vi "Event Handler.vi"(0 "Tamer in":refnum<class "Tamer.lvclass">, 5 "Event type":T1=enum."Message", 7 "Item Name":string, 9 "Data":variant, 11 "error in (no error)":errorcluster) -> (4 "Tamer out":refnum<class "Tamer.lvclass">, 15 "error out":errorcluster)   [LabVIEW 2020, in "Tamer.lvlib" / "Tamer.lvclass"]
doc: "This VI is the event handler of the uService: every time an event is triggered to the uService, this VI is called.\nNote: here you can access the Actor/Class data, but it will be the one coming out from Init. You cannot modify the values.\nThree different events are supported:\nI) Button Pressed: get called on a GUI button pressed. Item Name is the name (label) of the button, Data is empty.\nII) Shared Variable Updated: get called when a SV you subscribed to is updated. Item Name is the name of the SV, and Data is the value (note: you need to convert it to the proper type).\nIII) Message: get called every time a user event is generated using Send Message to Event Handler. The values of Item Name and Data are the one given to the Send Message to Event Handler.\nIV) Ready to launch?: this frame get called every time a new Run is initiated. Each uService is responsible of performing a self check before giving back the green light for the Run to start."
uses:
  Tamer.lvclass
  TALOS/TALOS_PPL.lvlibp/Father of all uServices/Father of all uServices/Event Handler Items.ctl
  Tamer Consumer Case Selector.ctl
  TALOS/TALOS_PPL.lvlibp/Support VIs/Go-NoGo.ctl
  Run Utilities/TypeDefs/Messages/Monkey Status Message.ctl
  Run Utilities/TypeDefs/Monkey Status.ctl
  Run Utilities/Schedule/Schedule.lvclass
  Run Utilities/TypeDefs/Messages/Script Checker Message.ctl
  Run Utilities/TypeDefs/Script Checker Result.ctl
  Run Utilities/TypeDefs/Messages/Banana Message.ctl
  Run Utilities/TypeDefs/Return Code.ctl
  Tamer.lvclass/Tamer.ctl
  TALOS/TALOS_PPL.lvlibp/Guardian/Guardian/Requests.ctl
  Open Debug Window.vi
  TALOS/TALOS_PPL.lvlibp/Father of all uServices/Father of all uServices/Father of all uServices.lvclass
  TALOS/TALOS_PPL.lvlibp
  TALOS/TALOS_PPL.lvlibp/Guardian/Guardian/Guardian.lvclass
  Run Utilities/Run Utilities.lvlib
  C:/LabVIEW Code/CIRCUS/TALOS/TALOS_PPL.lvlibp/Father of all uServices/Father of all uServices/Father of all uServices.lvclass
  C:/LabVIEW Code/CIRCUS/TALOS/TALOS_PPL.lvlibp/Ancestor/Ancestor/Ancestor.lvclass
  C:/LabVIEW Code/CIRCUS/TALOS/Actor Framework.lvlibp/1abvi3w/vi.lib/ActorFramework/Actor/Actor.lvclass
  C:/LabVIEW Code/CIRCUS/CIRCUS uServices et al/Tamer/Tamer.lvclass
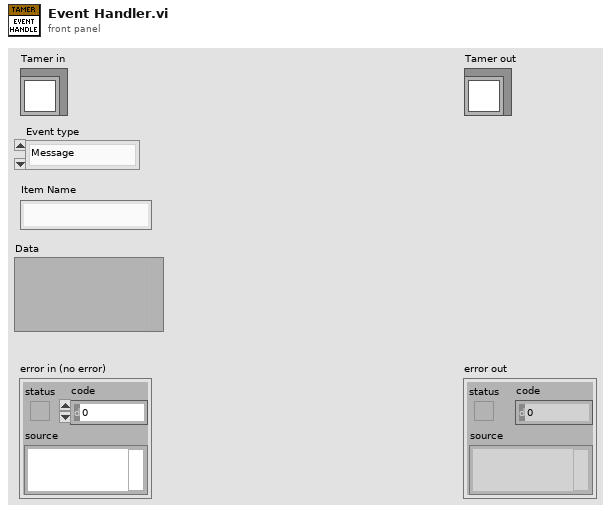
[diagram p1: front panel]
types:
  T1 = typedef "TALOS_PPL.lvlibp/Father of all uServices.lvlib/Father of all uServices.lvclass/Event Handler Items.ctl" = enum16{"Button Pressed", "Message", "Ready to launch?", "Safe Mode", "Start RUN", "Stop RUN"}
  T2 = typedef "Tamer.lvlib/Tamer.lvclass/Tamer Consumer Case Selector.ctl" = enum16{"New schedule", "Initiate RUN", "Parse Schedules", "Script Checker", "Banana after Quality Check", "Update Crit Lvl", "Propagate Banana", "Reply from Guardian", "Reply from uService", "Timeout of RUN", "uService Replies Check", "Update from Monkey", "Monkey Died", "Reschedule", "Rerun", "Stop DAQ", "Stop Schedule", "Skip Run", "Kill Process", "Update GV", "Append"}
  T3 = enum32{"Invalid", "Standard", "Closed", "Hidden", "Minimized", "Maximized"}
  T4 = typedef "TALOS_PPL.lvlibp/Go-NoGo.ctl" = cluster{"ID":string, "Status":bool, "Data":string[], "GUID":string}
  T5 = typedef "Run Utilities.lvlib/Monkey Status Message.ctl" = cluster{"Monkey ID":string, "Monkey Status":T6, "Scripts left":u32, "ETA":string, "Current Action":string, "Report from previous RUNs":string, "Skipped RUNs":refnum<class "Schedule.lvclass">}
  T6 = typedef "Run Utilities.lvlib/Monkey Status.ctl" = enum16{"Init", "Paused", "Ongoing", "Stopped", "Finished (no errors)", "Finished (with errors)"}
  T7 = typedef "Run Utilities.lvlib/Script Checker Message.ctl" = cluster{"Monkey ID":string, "Script Checker Result":T8}
  T8 = typedef "Run Utilities.lvlib/Script Checker Result.ctl" = enum16{"Passed", "Failed", "Empty"}
  T9 = typedef "Run Utilities.lvlib/Return Code.ctl" = enum16{"All Good", "Retry", "Skip", "Skip All", "ABORT"}
  T10 = typedef "Run Utilities.lvlib/Banana Message.ctl" = cluster{"FPGA Name":string, "Return Code":T9}
  T11 = typedef "TALOS_PPL.lvlibp/Guardian.lvlib/Guardian.lvclass/Requests.ctl" = enum16{"Ready to Launch", "Start RUN", "Stop RUN", "Update DAQ Params", "Update Error Listbox", "Update Run Status", "Update Kasli Log", "Run Stopped with Errors", "Switch uS View"}
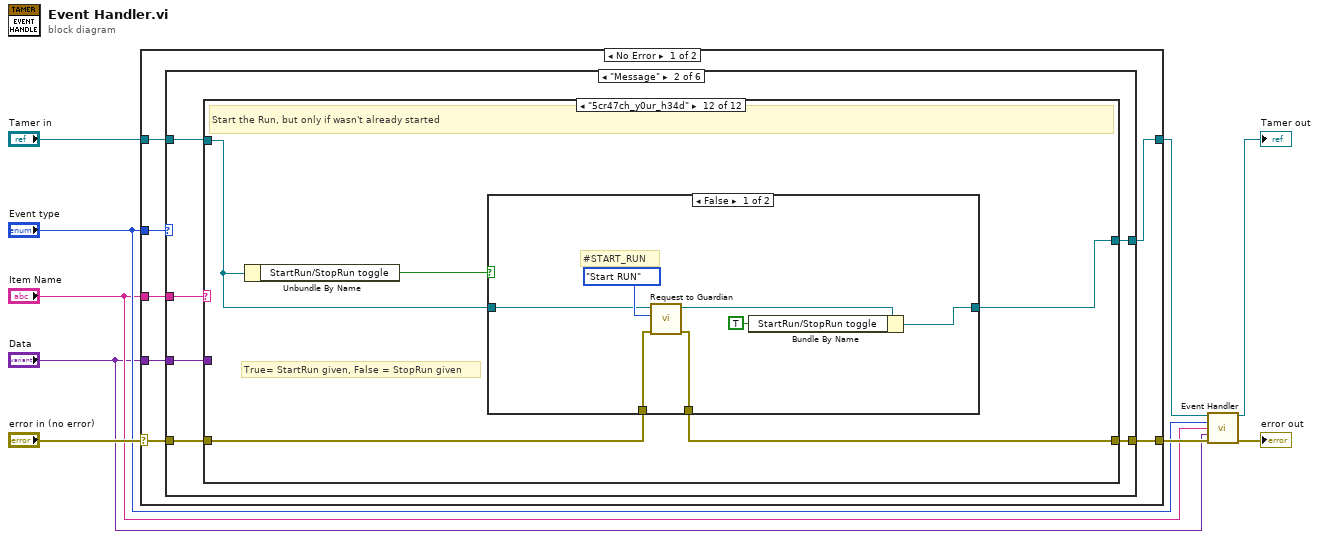
[diagram p0: block diagram]
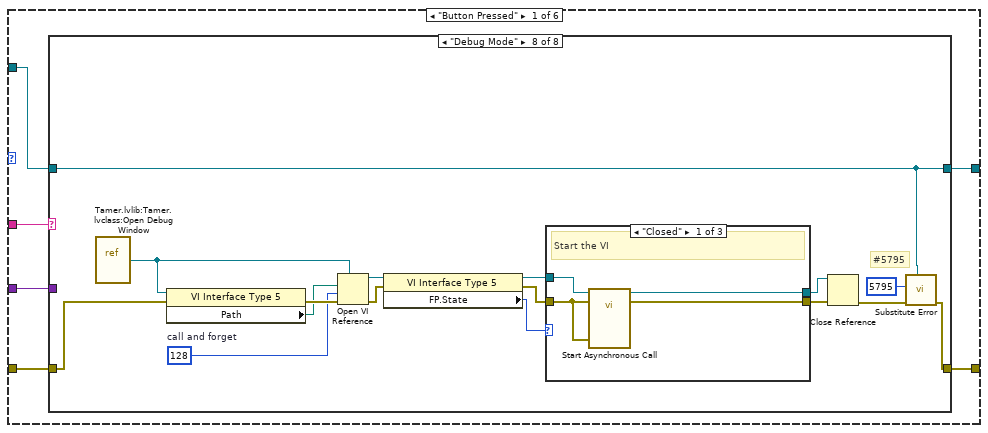
[diagram p2: hidden frame]
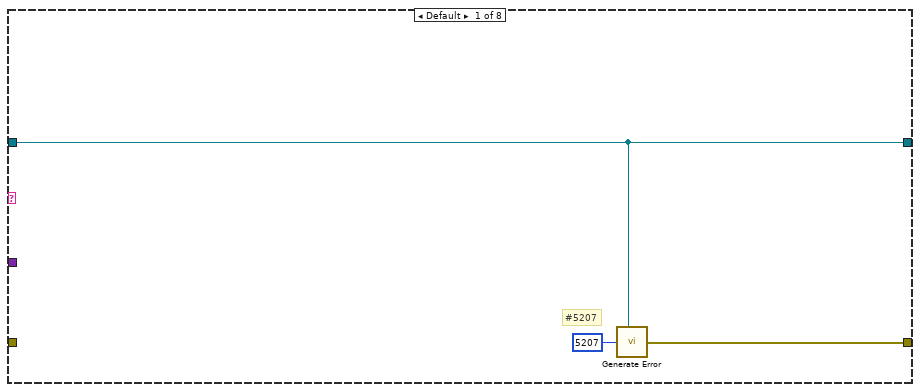
[diagram p3: hidden frame]
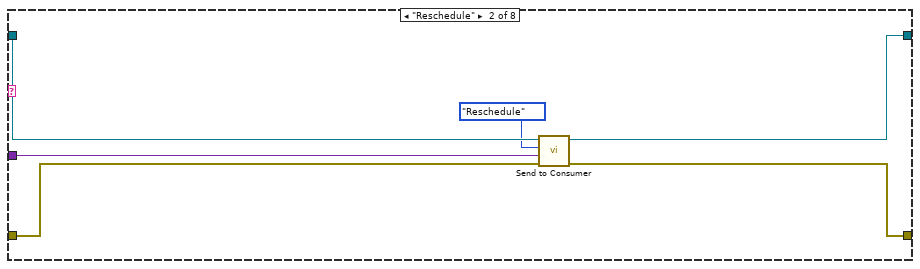
[diagram p4: hidden frame]
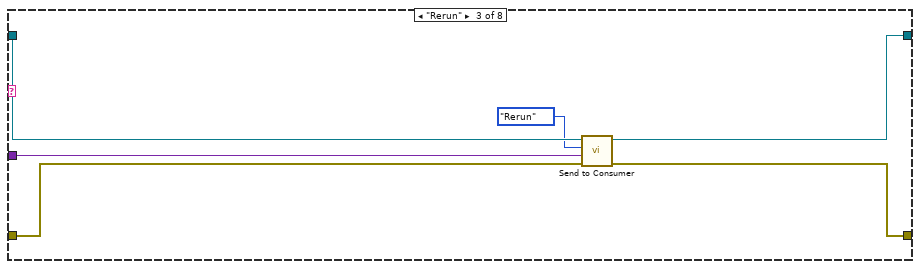
[diagram p5: hidden frame]
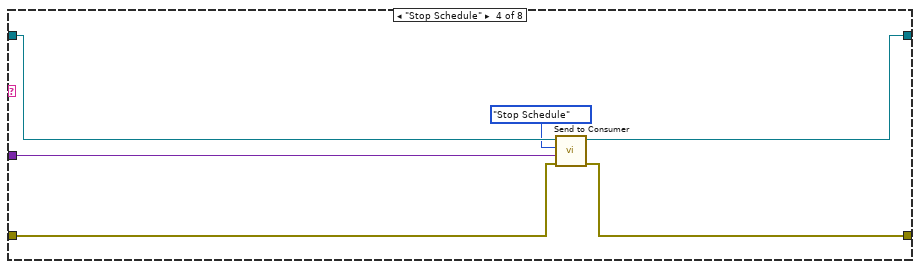
[diagram p6: hidden frame]
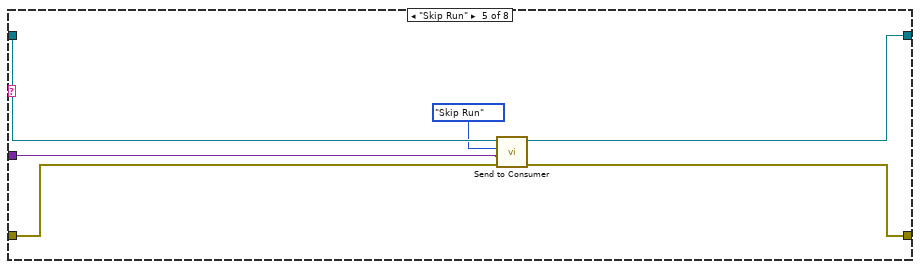
[diagram p7: hidden frame]
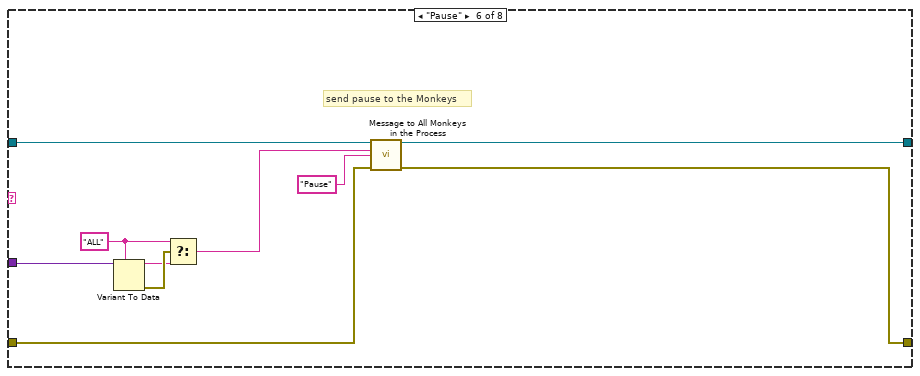
[diagram p8: hidden frame]
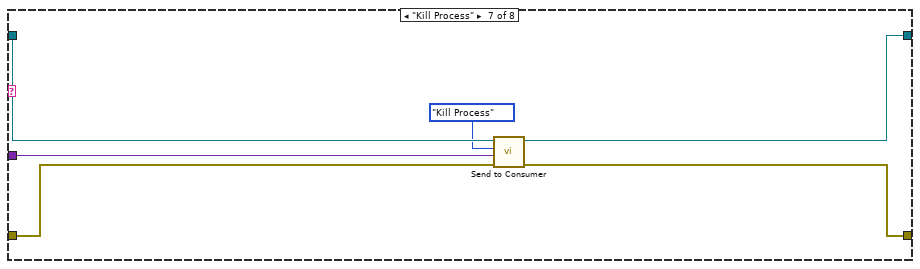
[diagram p9: hidden frame]
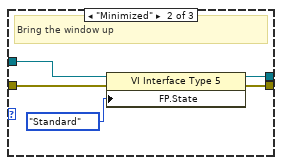
[diagram p10: hidden frame]
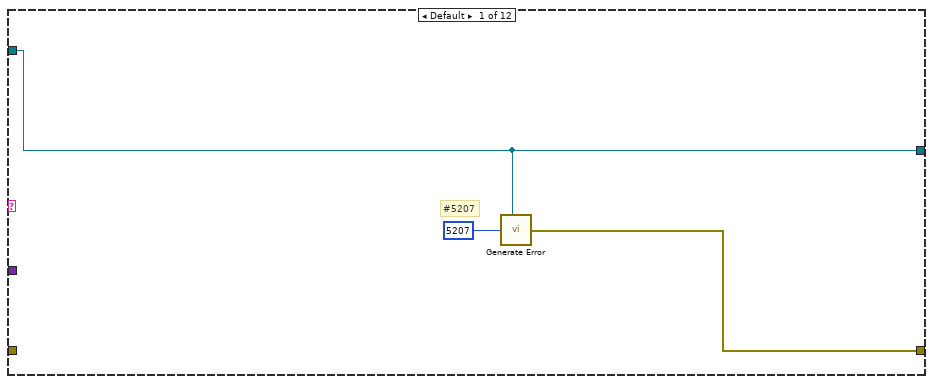
[diagram p12: hidden frame]
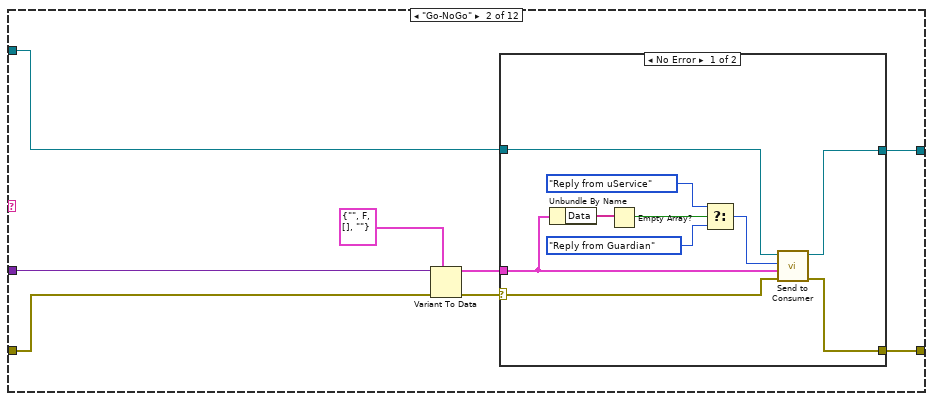
[diagram p13: hidden frame]
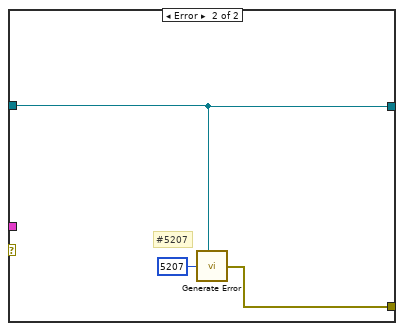
[diagram p14: hidden frame]
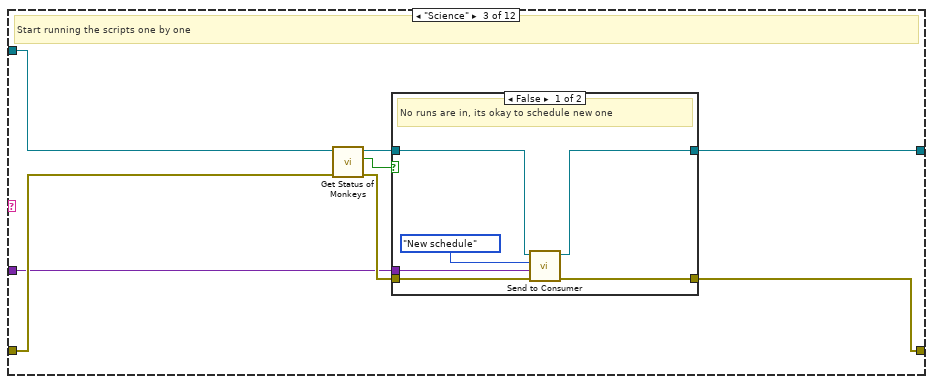
[diagram p15: hidden frame]
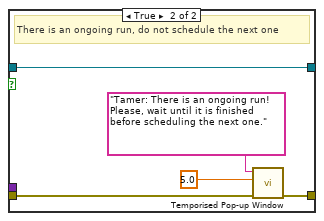
[diagram p16: hidden frame]
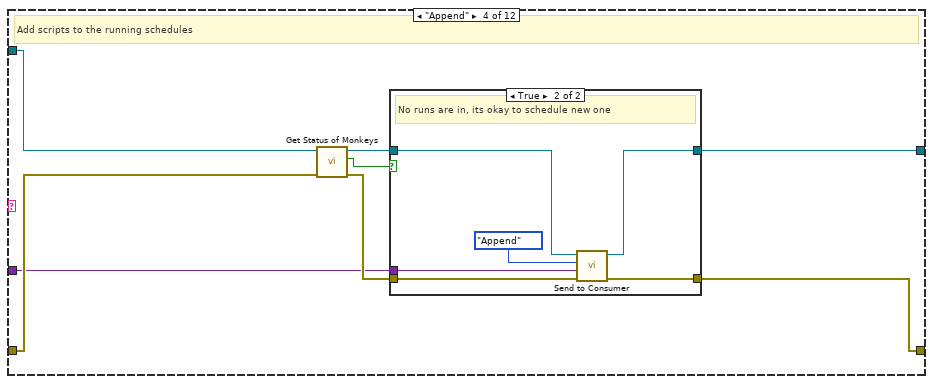
[diagram p17: hidden frame]
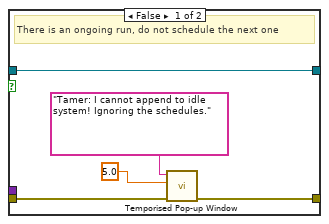
[diagram p18: hidden frame]
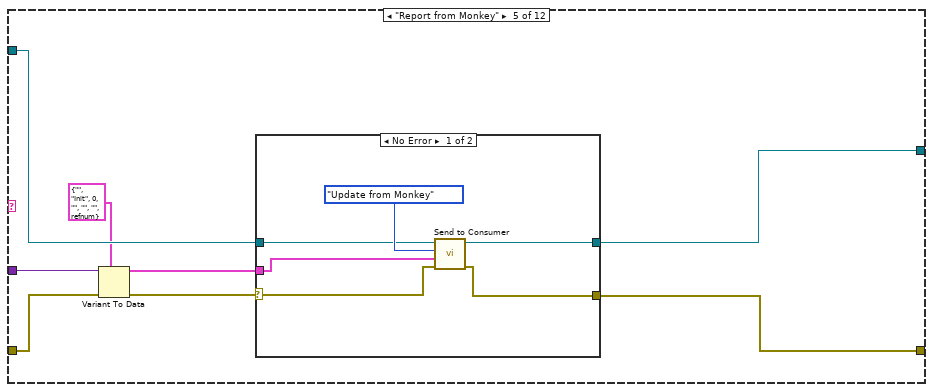
[diagram p19: hidden frame]
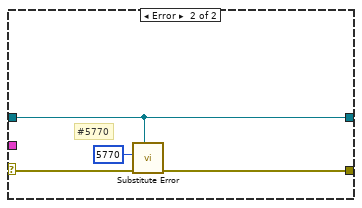
[diagram p20: hidden frame]
diagram:
  n1 = case shown="No Error" "error in (no error)" {
    selector: "error in (no error)" -> [w14 w337]
    tunnel: [w15 w337] -> w7
    tunnel: [w11 w336] -> w4
    tunnel: "Tamer in" -> [w10 w336]
    tunnel: "Event type" -> [w16 _]
    tunnel: "Item Name" -> [w13 _]
    tunnel: "Data" -> [w12 _]
    frame No Error {
      n2 = case shown="\"Message\"" w16 {
        tunnel: [w22 w94 w314 w323 w328 w335] -> w15
        tunnel: w14 -> [w19 w98 w315 w325 w329 w333]
        tunnel: w13 -> [w20 w97 _ _ _ _]
        tunnel: w10 -> [w21 w95 w313 w320 w330 w334]
        tunnel: w12 -> [w17 w96 w311 _ _ _]
        tunnel: [w18 w93 w310 w322 w326 w331] -> w11
        frame "Button Pressed" {
          n3 = case shown="\"Debug Mode\"" w20 {
            tunnel: w19 -> [_ w26 w32 w39 w45 w56 w63 w77]
            tunnel: [w24 w30 w35 w42 w46 w55 w60 w66] -> w22
            tunnel: w21 -> [w23 w31 w37 w43 w49 w58 w65 w67]
            tunnel: [w23 w28 w34 w41 w47 w57 w61 w67] -> w18
            tunnel: w17 -> [_ w27 w33 w38 w44 w54 w62 _]
            frame Default {
              # "#5207"
              n4 = call "Generate Error.vi"("Class"=w23, "Error Code"=5207) -> ("error out"=w24:errorcluster)  [unwired: 5 in]
            }
            frame "Reschedule" {
              n5 = call "Send to Consumer.vi"("error in (no error)"=w26, "Data"=w27, "Case ID"=Tamer_Consumer_Case_Selector."Reschedule" ("Monkey Consumer Case Selector"), "uService Template in"=w31) -> ("error out"=w30:errorcluster, "uService Template out"=w28:refnum<class "Tamer.lvclass">)  [unwired: 6 in]
            }
            frame "Rerun" {
              n6 = call "Send to Consumer.vi"("error in (no error)"=w32, "Data"=w33, "Case ID"=Tamer_Consumer_Case_Selector."Rerun" ("Monkey Consumer Case Selector"), "uService Template in"=w37) -> ("error out"=w35:errorcluster, "uService Template out"=w34:refnum<class "Tamer.lvclass">)  [unwired: 6 in]
            }
            frame "Stop Schedule" {
              n7 = call "Send to Consumer.vi"("error in (no error)"=w39, "Data"=w38, "Case ID"=Tamer_Consumer_Case_Selector."Stop Schedule" ("Monkey Consumer Case Selector"), "uService Template in"=w43) -> ("error out"=w42:errorcluster, "uService Template out"=w41:refnum<class "Tamer.lvclass">)  [unwired: 6 in]
            }
            frame "Skip Run" {
              n8 = call "Send to Consumer.vi"("error in (no error)"=w45, "Data"=w44, "Case ID"=Tamer_Consumer_Case_Selector."Skip Run" ("Monkey Consumer Case Selector"), "uService Template in"=w49) -> ("error out"=w46:errorcluster, "uService Template out"=w47:refnum<class "Tamer.lvclass">)  [unwired: 6 in]
            }
            frame "Pause" {
              w53 = "ALL"
              # "send pause to the Monkeys"
              n9 = Variant To Data(type=w53, Variant=w54) -> (data=w52:string, error out=w59:errorcluster)  [unwired: 1 in]
              n10 = Select(t=w53, s=w59, f=w52) -> (s? t:f=w51:string)
              n11 = call-dynamic "Message to All Monkeys in the Process.vi"("Tamer in"=w58, "Process ID"=w51, "Message"="Pause" ("Process ID"), "error in (no error)"=w56) -> ("Tamer out"=w57:refnum<class "Tamer.lvclass">, "error out"=w55:errorcluster)  [unwired: 10 in]
            }
            frame "Kill Process" {
              n12 = call "Send to Consumer.vi"("error in (no error)"=w63, "Data"=w62, "Case ID"=Tamer_Consumer_Case_Selector."Kill Process" ("Monkey Consumer Case Selector"), "uService Template in"=w65) -> ("error out"=w60:errorcluster, "uService Template out"=w61:refnum<class "Tamer.lvclass">)  [unwired: 6 in]
            }
            frame "Debug Mode" {
              w78 = 128  # call and forget
              # "#5795"
              n13 = vi-ref "Tamer.lvlib:Tamer.lvclass:Open Debug Window.vi"() -> (w76:refnum<vi>)
              n14 = property class="VI Interface Type 5"(reference=w76, error in=w77) -> (error out=w81:errorcluster, "Path"=w80:path)  [unwired: 1 out]
              n15 = Open VI Reference(type specifier VI Refnum (for type only)=w76, vi path=w80, options=w78, error in (no error)=w81) -> (vi reference=w79:refnum<vi>, error out=w74:errorcluster)  [unwired: 2 in]
              n16 = property class="VI Interface Type 5"(reference=w79, error in=w74) -> (reference out=w75:refnum<vi>, error out=w73:errorcluster, "FP.State"=w72:T3)
              n17 = case shown="\"Closed\"" w72 {
                tunnel: w75 -> [w85 w88 w92]
                tunnel: w73 -> [w84 w90 w91]
                tunnel: [w83 w89 w91] -> w69
                tunnel: [w82 w86 w92] -> w68
                frame "Closed" {
                  # "Start the VI"
                  n18 = call-by-ref "Start Asynchronous Call"(reference=w85, error in=w84, 8:"error in (no error)"=w84) -> (reference out=w82:refnum<vi>, error out=w83:errorcluster)  [unwired: 10 in, 1 out]
                }
                frame "Minimized" {
                  # "Bring the window up"
                  n19 = property class="VI Interface Type 5"(reference=w88, error in=w90, "FP.State"=T3."Standard" ("Front Panel Window:State")) -> (reference out=w86:refnum<vi>, error out=w89:errorcluster)
                }
                frame Default {
                  # "Either running or something is worng, do nothing"
                }
              }
              n20 = Close Reference(reference=w68, error in (no error)=w69) -> (error out=w71:errorcluster)
              n21 = call "Substitute Error.vi"("LabVIEW Object"=w67, "error in (no error)"=w71, "Error Code"=5795) -> ("error out"=w66:errorcluster)  [unwired: 8 in]
            }
          }
        }
        frame "Message" {
          n22 = case shown="\"5cr47ch_y0ur_h34d\"" w97 {
            tunnel: w98 -> [_ w108 w130 w149 w167 w180 w191 w208 w246 w266 w283 w300]
            tunnel: w96 -> [_ w105 w128 w147 w168 w181 w190 w210 w242 w265 w288 _]
            tunnel: w95 -> [w99 w103 w126 w142 w165 w184 w187 w204 w247 w264 w285 w297]
            tunnel: [w100 w109 w127 w146 w162 w183 w185 w205 w243 w267 w278 w299] -> w94
            tunnel: [w99 w102 w123 w143 w161 w179 w186 w203 w252 w263 w286 w298] -> w93
            frame Default {
              # "#5207"
              n23 = call "Generate Error.vi"("Class"=w99, "Error Code"=5207) -> ("error out"=w100:errorcluster)  [unwired: 5 in]
            }
            frame "Go-NoGo" {
              n24 = Variant To Data(error in=w108, type=T4 {"ID"="", "Status"=FALSE, "Data"=[], "GUID"=""} ("Go-NoGo"), Variant=w105) -> (data=w104:T4, error out=w106:errorcluster)
              n25 = case shown="No Error" w106 {
                selector: w106 -> [w117 _]
                tunnel: [w119 w121] -> w109
                tunnel: w104 -> [w114 _]
                tunnel: w103 -> [w116 w120]
                tunnel: [w115 w120] -> w102
                frame No Error {
                  n26 = Unbundle By Name(w114) -> ("Data"=w118:string[])
                  n27 = Empty Array?(array=w118) -> (empty?=w113:bool)
                  n28 = Select(t=Tamer_Consumer_Case_Selector."Reply from uService" ("Monkey Consumer Case Selector"), s=w113, f=Tamer_Consumer_Case_Selector."Reply from Guardian" ("Monkey Consumer Case Selector")) -> (s? t:f=w110:T2)
                  n29 = call "Send to Consumer.vi"("error in (no error)"=w117, "Data"=w114, "Case ID"=w110, "uService Template in"=w116) -> ("error out"=w119:errorcluster, "uService Template out"=w115:refnum<class "Tamer.lvclass">)  [unwired: 6 in]
                }
                frame Error {
                  # "#5207"
                  n30 = call "Generate Error.vi"("Class"=w120, "Error Code"=5207) -> ("error out"=w121:errorcluster)  [unwired: 5 in]
                }
              }
            }
            frame "Science" {
              # "Start running the scripts one by one"
              n31 = call-dynamic "Get Status of Monkeys.vi"("error in (no error)"=w130, "Tamer in"=w126) -> ("error out"=w129:errorcluster, "Anything running?"=w124:bool, "Tamer out"=w125:refnum<class "Tamer.lvclass">)  [unwired: 7 in]
              n32 = case shown="False" w124 {
                tunnel: w128 -> [w134 _]
                tunnel: [w136 w138] -> w127
                tunnel: w125 -> [w131 w137]
                tunnel: w129 -> [w133 w141]
                tunnel: [w132 w137] -> w123
                frame False {
                  # "No runs are in, its okay to schedule new one"
                  n33 = call "Send to Consumer.vi"("error in (no error)"=w133, "Data"=w134, "Case ID"=Tamer_Consumer_Case_Selector."New schedule" ("Monkey Consumer Case Selector"), "uService Template in"=w131) -> ("error out"=w136:errorcluster, "uService Template out"=w132:refnum<class "Tamer.lvclass">)  [unwired: 6 in]
                }
                frame True {
                  # "There is an ongoing run, do not schedule the next one"
                  n34 = call "Temporised Pop-up Window.vi"("error in (no error)"=w141, "Timeout"=5.0, "Text"="Tamer: There is an ongoing run! Please, wait until it is finished before scheduling the next one.") -> ("error out"=w138:errorcluster)  [unwired: 8 in]
                }
              }
            }
            frame "Append" {
              # "Add scripts to the running schedules"
              n35 = call-dynamic "Get Status of Monkeys.vi"("error in (no error)"=w149, "Tamer in"=w142) -> ("error out"=w148:errorcluster, "Anything running?"=w144:bool, "Tamer out"=w145:refnum<class "Tamer.lvclass">)  [unwired: 7 in]
              n36 = case shown="True" w144 {
                tunnel: w147 -> [_ w157]
                tunnel: [w151 w159] -> w146
                tunnel: w145 -> [w150 w160]
                tunnel: w148 -> [w154 w156]
                tunnel: [w150 w155] -> w143
                frame False {
                  # "There is an ongoing run, do not schedule the next one"
                  n37 = call "Temporised Pop-up Window.vi"("error in (no error)"=w154, "Timeout"=5.0, "Text"="Tamer: I cannot append to idle system! Ignoring the schedules.") -> ("error out"=w151:errorcluster)  [unwired: 8 in]
                }
                frame True {
                  # "No runs are in, its okay to schedule new one"
                  n38 = call "Send to Consumer.vi"("error in (no error)"=w156, "Data"=w157, "Case ID"=Tamer_Consumer_Case_Selector."Append" ("Monkey Consumer Case Selector"), "uService Template in"=w160) -> ("error out"=w159:errorcluster, "uService Template out"=w155:refnum<class "Tamer.lvclass">)  [unwired: 6 in]
                }
              }
            }
            frame "Report from Monkey" {
              n39 = Variant To Data(error in=w167, type=T5 {"Monkey ID"="", "Monkey Status"=enum."Init", "Scripts left"=0, "ETA"="", "Current Action"="", "Report from previous RUNs"="", "Skipped RUNs"=refnum} ("Monkey Status Message"), Variant=w168) -> (data=w164:T5, error out=w166:errorcluster)
              n40 = case shown="No Error" w166 {
                selector: w166 -> [w173 w178]
                tunnel: w165 -> [w172 w175]
                tunnel: w164 -> [w171 _]
                tunnel: [w170 w176] -> w162
                tunnel: [w169 w175] -> w161
                frame No Error {
                  n41 = call "Send to Consumer.vi"("error in (no error)"=w173, "Data"=w171, "Case ID"=Tamer_Consumer_Case_Selector."Update from Monkey" ("Monkey Consumer Case Selector"), "uService Template in"=w172) -> ("error out"=w170:errorcluster, "uService Template out"=w169:refnum<class "Tamer.lvclass">)  [unwired: 6 in]
                }
                frame Error {
                  # "#5770"
                  n42 = call "Substitute Error.vi"("LabVIEW Object"=w175, "error in (no error)"=w178, "Error Code"=5770) -> ("error out"=w176:errorcluster)  [unwired: 8 in]
                }
              }
            }
            frame "I'm DEAD" {
              # "Monkey was killed with the STOP button (or harakiri)"
              n43 = call "Send to Consumer.vi"("error in (no error)"=w180, "Data"=w181, "Case ID"=Tamer_Consumer_Case_Selector."Monkey Died" ("Monkey Consumer Case Selector"), "uService Template in"=w184) -> ("error out"=w183:errorcluster, "uService Template out"=w179:refnum<class "Tamer.lvclass">)  [unwired: 6 in]
            }
            frame "Script Checker" {
              # "Synced Monkey Performed Script Check"
              n44 = Variant To Data(error in=w191, type=T7 {"Monkey ID"="", "Script Checker Result"=enum."Passed"} ("Message"), Variant=w190) -> (data=w188:T7, error out=w189:errorcluster)
              n45 = case shown="No Error" w189 {
                selector: w189 -> [w194 w200]
                tunnel: [w198 w201] -> w185
                tunnel: w187 -> [w197 w199]
                tunnel: w188 -> [w196 _]
                tunnel: [w193 w199] -> w186
                frame No Error {
                  n46 = call "Send to Consumer.vi"("error in (no error)"=w194, "Data"=w196, "Case ID"=Tamer_Consumer_Case_Selector."Script Checker" ("Monkey Consumer Case Selector"), "uService Template in"=w197) -> ("error out"=w198:errorcluster, "uService Template out"=w193:refnum<class "Tamer.lvclass">)  [unwired: 6 in]
                }
                frame Error {
                  # "#5757"
                  n47 = call "Substitute Error.vi"("LabVIEW Object"=w199, "error in (no error)"=w200, "Error Code"=5757) -> ("error out"=w201:errorcluster)  [unwired: 8 in]
                }
              }
            }
            frame "B4n4n4" {
              # "Script finished. Send it to Monkey for the quality check"
              n48 = Variant To Data(error in=w208, type=string[] [], Variant=w210) -> (data=w207:string[], error out=w206:errorcluster)
              n49 = case shown="No Error" w206 {
                selector: w206 -> [w233 w241]
                tunnel: w207 -> [w237 _]
                tunnel: [w217 w240] -> w205
                tunnel: w204 -> [w231 w238]
                tunnel: [w228 w238] -> w203
                frame No Error {
                  w211 = "Quality Check" ("Message")
                  # "#5752\nB4n4n4"
                  n50 = Index Array(array=w237) -> (element #1=w218:string, element #2=w234:string)  [unwired: 2 in]
                  n51 = Decimal String To Number(string=w234, default (0L)=3) -> (number=w235:i32)  [unwired: 1 in, 1 out]
                  n52 = Variant To Data(error in=w233, type=Return_Code."Skip All" ("Return Code"), Variant=w235) -> (data=w227:T9, error out=w230:errorcluster)
                  n53 = call-dynamic "Get Monkey ID From FPGA Name.vi"("error in (no error)"=w230, "FPGA Name"=w218, "Tamer in"=w231) -> ("error out"=w226:errorcluster, "Monkey ID"=w221:string, "Tamer out"=w225:refnum<class "Tamer.lvclass">)  [unwired: 6 in]
                  n54 = Bundle(cluster=T10 {"FPGA Name"="", "Return Code"=enum."All Good"} ("Cluster"), "FPGA Name"=w218, "Return Code"=w227) -> (w216:T10)
                  n55 = call "Message to uService.vi"("Father of all uServices in"=w225, "uService ID"=w221, "Message"=w211, "Data"=w216, "error in (no error)"=w226) -> ("Father of all uServices out"=w215:refnum<class "Tamer.lvclass">, "error out"=w222:errorcluster)  [unwired: 9 in]
                  n56 = Concatenate Strings(w211, " to " ("string"), w221) -> (w220:string)
                  n57 = call "FPGA informative error on return.vi"("Message"=w216, "Class in"=w215) -> ("error out"=w213:errorcluster)  [unwired: 9 in]
                  n58 = call-dynamic "Update Action History.vi"("error in (no error)"=w222, "Action"=w220, "Tamer in"=w215) -> ("error out"=w214:errorcluster, "Tamer out"=w228:refnum<class "Tamer.lvclass">)  [unwired: 7 in]
                  n59 = Merge Errors(w214, w213) -> (w212:errorcluster)
                  n60 = call "Substitute Error.vi"("LabVIEW Object"=w228, "error in (no error)"=w212, "Error Code"=5752, "Optional String"="Tamer doesn't know who sent B4n4n4") -> ("error out"=w217:errorcluster)  [unwired: 7 in]
                }
                frame Error {
                  # "#5789"
                  n61 = call "Substitute Error.vi"("LabVIEW Object"=w238, "error in (no error)"=w241, "Error Code"=5789) -> ("error out"=w240:errorcluster)  [unwired: 8 in]
                }
              }
            }
            frame "Quality Check - result" {
              n62 = Variant To Data(type=T10 {"FPGA Name"="", "Return Code"=enum."All Good"} ("Cluster"), Variant=w242) -> (data=w248:T10, error out=w249:errorcluster)  [unwired: 1 in]
              n63 = case shown="No Error" w249 {
                tunnel: w248 -> [w257 _]
                tunnel: w247 -> [w260 w261]
                tunnel: [w255 _] -> w244
                tunnel: [w256 w261] -> w253
                frame No Error {
                  # "Check if quality of run was passed. If not, give an error to have that information in the error log"
                  n64 = Unbundle By Name(w257) -> ("FPGA Name"=w258:string)
                  n65 = Concatenate Strings("Received the quality check from ", w258) -> (w254:string)
                  n66 = call-dynamic "Update Action History.vi"("Action"=w254, "Tamer in"=w260) -> ("error out"=w255:errorcluster, "Tamer out"=w256:refnum<class "Tamer.lvclass">)  [unwired: 8 in]
                }
                frame Error {
                  # "Wrong format, this is delt with in the consumer"
                }
              }
              n67 = call "Send to Consumer.vi"("error in (no error)"=w246, "Data"=w242, "Case ID"=Tamer_Consumer_Case_Selector."Banana after Quality Check" ("Monkey Consumer Case Selector"), "uService Template in"=w253) -> ("error out"=w245:errorcluster, "uService Template out"=w252:refnum<class "Tamer.lvclass">)  [unwired: 6 in]
              n68 = Merge Errors(w245, w244) -> (w243:errorcluster)
            }
            frame "570prun" {
              # "True= StartRun given, False = StopRun given"
              # "Issue Stop Run to all the uServices and Guardians."
              n69 = Unbundle By Name(w264) -> ("StartRun/StopRun toggle"=w262:bool)
              n70 = case shown="True" w262 {
                tunnel: [w269 w277] -> w267
                tunnel: w266 -> [w269 w276]
                tunnel: w265 -> [_ w275]
                tunnel: w264 -> [w268 w273]
                tunnel: [w268 w271] -> w263
                frame False {
                  # "Do nothing"
                }
                frame True {
                  # "#STOP_RUN"
                  n71 = call "Request to Guardian.vi"("error in (no error)"=w276, "Data"=w275, "Requests"=Requests."Stop RUN", "Father of all uServices in"=w273) -> ("error out"=w277:errorcluster, "Father of all uServices out"=w272:refnum<class "Tamer.lvclass">)  [unwired: 6 in]
                  n72 = Bundle By Name(cluster=w272, "StartRun/StopRun toggle"=FALSE) -> (w271:refnum<class "Tamer.lvclass">)
                }
              }
            }
            frame "Error Criticality" {
              # "Error occured when running a script"
              n73 = call-dynamic "Get Status of Monkeys.vi"("error in (no error)"=w283, "Tamer in"=w285) -> ("error out"=w289:errorcluster, "Anything running?"=w281:bool, "Tamer out"=w284:refnum<class "Tamer.lvclass">)  [unwired: 7 in]
              n74 = Not(x=w289) -> (.not. x?=w282:bool)
              n75 = Select(t=w281, s=w282, f=TRUE) -> (s? t:f=w279:bool)
              n76 = case shown="True" w279 {
                tunnel: w288 -> [_ w294]
                tunnel: [_ w293] -> w287
                tunnel: [w290 w291] -> w286
                tunnel: w284 -> [w290 w295]
                frame False {
                }
                frame True {
                  n77 = call "Send to Consumer.vi"("Data"=w294, "Case ID"=Tamer_Consumer_Case_Selector."Update Crit Lvl" ("Monkey Consumer Case Selector"), "uService Template in"=w295) -> ("error out"=w293:errorcluster, "uService Template out"=w291:refnum<class "Tamer.lvclass">)  [unwired: 7 in]
                }
              }
              n78 = Merge Errors(w287, w289) -> (w278:errorcluster)
            }
            frame "5cr47ch_y0ur_h34d" {
              # "True= StartRun given, False = StopRun given"
              # "Start the Run, but only if wasn't already started"
              n79 = Unbundle By Name(w297) -> ("StartRun/StopRun toggle"=w296:bool)
              n80 = case shown="False" w296 {
                tunnel: w300 -> [w307 w308]
                tunnel: [w306 w308] -> w299
                tunnel: [w303 w309] -> w298
                tunnel: w297 -> [w301 w309]
                frame False {
                  # "#START_RUN"
                  n81 = call "Request to Guardian.vi"("error in (no error)"=w307, "Requests"=Requests."Start RUN", "Father of all uServices in"=w301) -> ("error out"=w306:errorcluster, "Father of all uServices out"=w305:refnum<class "Tamer.lvclass">)  [unwired: 7 in]
                  n82 = Bundle By Name(cluster=w305, "StartRun/StopRun toggle"=TRUE ("StartRun already given?")) -> (w303:refnum<class "Tamer.lvclass">)
                }
                frame True {
                  # "Do nothing"
                }
              }
            }
          }
        }
        frame "Ready to launch?" {
          # "Don't remove this wire!"
          # "Just give green light: \"Cogito ergo sum\" - Volpe"
          n83 = call-dynamic "Go-NoGo.vi"("error in (no error)"=w315, "Go-NoGo Data"=w311, "Go?"=TRUE, "Father of all uServices in"=w313) -> ("error out"=w314:errorcluster, "Father of all uServices out"=w310:refnum<class "Tamer.lvclass">)  [unwired: 6 in]
        }
        frame "Safe Mode" {
          n84 = call-dynamic "Update Monkeys Status.vi"("In ALL?"=TRUE, "Status"=Monkey_Status."Finished (with errors)", "Tamer in"=w320) -> ("error out"=w318:errorcluster, "Tamer out"=w321:refnum<class "Tamer.lvclass">)  [unwired: 7 in]
          n85 = call "Send to Consumer.vi"("Case ID"=Tamer_Consumer_Case_Selector."Stop Schedule" ("Monkey Consumer Case Selector"), "uService Template in"=w321) -> ("error out"=w319:errorcluster, "uService Template out"=w322:refnum<class "Tamer.lvclass">)  [unwired: 8 in]
          n86 = Merge Errors(w319, w318, w325) -> (w323:errorcluster)
        }
        frame "Start RUN" {
          n87 = call-dynamic "Update Action History.vi"("error in (no error)"=w329, "Action"="Start Run" ("GUI Item Name"), "Tamer in"=w330) -> ("error out"=w328:errorcluster, "Tamer out"=w326:refnum<class "Tamer.lvclass">)  [unwired: 7 in]
        }
        frame "Stop RUN" {
          n88 = call-dynamic "Update Action History.vi"("error in (no error)"=w333, "Action"="Experiment finished! Ending the script..." ("GUI Item Name"), "Tamer in"=w334) -> ("error out"=w335:errorcluster, "Tamer out"=w331:refnum<class "Tamer.lvclass">)  [unwired: 7 in]
        }
      }
    }
    frame Error {
    }
  }
  n89 = call-parent "Event Handler.vi"("uService Template in"=w4, "Event type"="Event type", "Item Name"="Item Name", "Data"="Data", "error in (no error)"=w7) -> ("uService Template out"=→"Tamer out":refnum<class "Tamer.lvclass">, "error out"=→"error out":errorcluster)  [unwired: 9 in]
